vi "Module Init.vi"(8 "error in (no error)":errorcluster, 11 "Sequencing in":refnum<class "Sequencing.lvclass">) -> (0 "error out":errorcluster, 3 "Sequencing out":refnum<class "Sequencing.lvclass">)   [LabVIEW 2020, in "VolatusSeq.lvlib" / "Sequencing.lvclass"]
uses:
  Sequencing.lvclass
  C:/dev/lv20CE/relink/lv-volatus/Volatus/Module/Module.lvclass
  Volatus/Message Registration.ctl
  Volatus/Module/Module.lvclass/Module.ctl
  Volatus/VolatusAPI/VolatusAPI.lvclass/VolatusAPI.ctl
  lv-http-server/HTTP Server/Server/Register Handler.vi
  SequencingHttpCtrlr/SequencingHttpCtrlr.lvclass
  C:/dev/lv20CE/relink/lv-http-server/HTTP Server/Handler/Handler.lvclass
  lv-vecto/Vecto/Vecto/Get HTTP.vi
  lv-http-server/HTTP Server/Server/Add Connection Handler.vi
  lv-http-server/HTTP Server/Server/Add Request Handler.vi
  lv-http-server/HTTP Server/Server/Add Route Handler.vi
  lv-http-server/HTTP Server/Server/Add Controller Handler.vi
  lv-http-server/HTTP Server/Server/Add Controller.vi
  lv-http-server/HTTP Server/Server/Add Response Handler.vi
  lv-http-server/HTTP Server/Server/Add Complete Handler.vi
  lv-http-server/HTTP Server/Server/Add Exception Handler.vi
  lv-http-server/HTTP Server/Connection Handler/Connection Handler.lvclass
  lv-http-server/HTTP Server/Request Handler/Request Handler.lvclass
  lv-http-server/HTTP Server/Route Handler/Route Handler.lvclass
  lv-http-server/HTTP Server/Controller Handler/Controller Handler.lvclass
  lv-http-server/HTTP Server/Controller/Controller.lvclass
  lv-http-server/HTTP Server/Response Handler/Response Handler.lvclass
  lv-http-server/HTTP Server/Complete Handler/Complete Handler.lvclass
  lv-http-server/HTTP Server/Exception Handler/Exception Handler.lvclass
  lv-http-server/HTTP Server/Handler/Handler.lvclass
  Sequencing.lvclass/Sequencing.ctl
  Volatus/Module/Module.lvclass
  Volatus/VolatusAPI/VolatusAPI.lvclass
  C:/dev/lv20CE/relink/lv-volatus/VolatusSeq/Sequencing/Sequencing.lvclass
  Volatus/Volatus.lvlib
  C:/dev/lv20CE/relink/lv-http-server/HTTP Server/Controller/Controller.lvclass
  C:/dev/lv20CE/relink/lv-volatus/VolatusSeq/SequencingHttpCtrlr/SequencingHttpCtrlr.lvclass
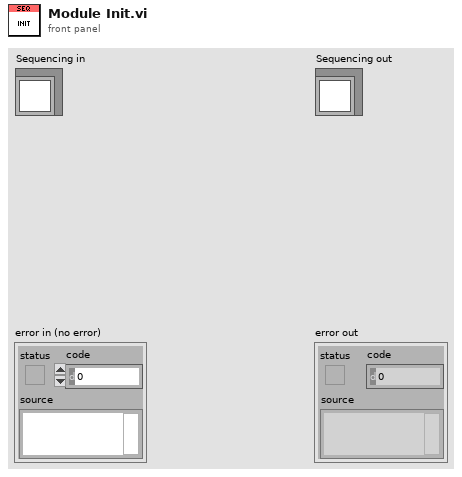
[diagram p1: front panel]
types:
  T1 = typedef "Volatus.lvlib/Message Registration.ctl" = cluster{"Message Type":string, "Message ID":string}
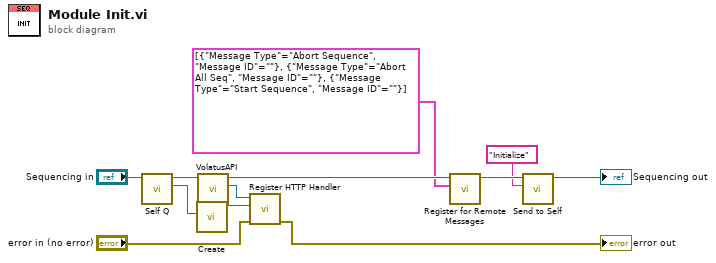
[diagram p0: block diagram]
diagram:
  n1 = call "Self Q.vi"("Module in"="Sequencing in") -> ("Self Q"=w8:refnum<class "MessageQ.lvclass">, "Module out"=w9:refnum<class "Sequencing.lvclass">)  [unwired: 9 in]
  n2 = call "Create.vi"("Msg Q"=w8) -> ("SequencingHttpCtrlr out"=w7:refnum<class "SequencingHttpCtrlr.lvclass">)  [unwired: 9 in, 1 out]
  n3 = call "VolatusAPI.vi"("Module in"=w9) -> ("VolatusAPI"=w10:refnum<class "VolatusAPI.lvclass">, "Module out"=w11:refnum<class "Sequencing.lvclass">)  [unwired: 9 in]
  n4 = call "Register HTTP Handler.vi"("error in (no error)"="error in (no error)", "Handler"=w7, "VolatusAPI in"=w10) -> ("error out"=→"error out":errorcluster)  [unwired: 7 in, 1 out]
  n5 = call "Register for Remote Messages.vi"("Messages"=T1[] [{"Message Type"="Abort Sequence", "Message ID"=""}, {"Message Type"="Abort All Seq", "Message ID"=""}, {"Message Type"="Start Sequence", "Message ID"=""}], "Module in"=w11) -> ("Module out"=w4:refnum<class "Sequencing.lvclass">)  [unwired: 8 in, 1 out]
  n6 = call "Send to Self.vi"("Message ID"="Initialize", "Module in"=w4) -> ("Module out"=→"Sequencing out":refnum<class "Sequencing.lvclass">)  [unwired: 8 in, 1 out]
